vi "Pi_Test_Pulses.vi"(10 "Pi/2 time":dbl=2e-09, 11 "Numeric":i32) -> (3 "x+y":dbl)   [LabVIEW 2024]
panel:
  out "x+y 2":dbl
  in  "clock_freq (MHz)":dbl=500.0
  in  "# of Instructions":u32=3
  in  "Path to spinapi.dll":path=path "C:/SpinCore/SpinAPI/lib/spinapi64.dll"
  in  "Instructions":T1(array[cluster])=[{"Instruct Data"=0, "Op Code"=0, "Flags"=[FALSE, TRUE, TRUE, FALSE, FALSE, FALSE, FALSE, FALSE, FALSE, FALSE, FALSE, FALSE, FALSE, FALSE, FALSE, FALSE, FALSE, FALSE, FALSE, FALSE, FALSE, FALSE, FALSE, TRUE], "Comments"="0", "Time (s)"=1e-07}, {"Instruct Data"=0, "Op Code"=0, "Flags"=[TRUE, TRUE, FALSE, TRUE, FALSE, FALSE, FALSE, FALSE, FALSE, FALSE, FALSE, FALSE, FALSE, FALSE, FALSE, FALSE, FALSE, FALSE, FALSE, FALSE, FALSE, FALSE, FALSE, FALSE], "Comments"="1", "Time (s)"=2e-06}, {"Instruct Data"=0, "Op Code"=6, "Flags"=[FALSE, TRUE, FALSE, FALSE, FALSE, FALSE, FALSE, FALSE, FALSE, FALSE, FALSE, FALSE, FALSE, FALSE, FALSE, FALSE, FALSE, FALSE, FALSE, FALSE, FALSE, FALSE, FALSE, FALSE], "Comments"="2", "Time (s)"=2e-06}, {"Instruct Data"=0, "Op Code"=6, "Flags"=[FALSE, TRUE, FALSE, FALSE, FALSE, FALSE, FALSE, FALSE, FALSE, FALSE, FALSE, FALSE, FALSE, FALSE, FALSE, FALSE, FALSE, FALSE, FALSE, FALSE, FALSE, FALSE, FALSE, FALSE], "Comments"="3", "Time (s)"=2e-06}, {"Instruct Data"=0, "Op Code"=6, "Flags"=[FALSE, TRUE, FALSE, FALSE, FALSE, FALSE, FALSE, FALSE, FALSE, FALSE, FALSE, FALSE, FALSE, FALSE, FALSE, FALSE, FALSE, FALSE, FALSE, FALSE, FALSE, FALSE, FALSE, FALSE], "Comments"="4", "Time (s)"=2e-06}, {"Instruct Data"=0, "Op Code"=6, "Flags"=[FALSE, FALSE, FALSE, FALSE, FALSE, FALSE, FALSE, FALSE, FALSE, FALSE, FALSE, FALSE, FALSE, FALSE, FALSE, FALSE, FALSE, FALSE, FALSE, FALSE, FALSE, FALSE, FALSE, FALSE], "Comments"="5", "Time (s)"=5e-06}, {"Instruct Data"=0, "Op Code"=6, "Flags"=[FALSE, TRUE, TRUE, FALSE, FALSE, FALSE, FALSE, FALSE, FALSE, FALSE, FALSE, FALSE, FALSE, FALSE, FALSE, FALSE, FALSE, FALSE, FALSE, FALSE, FALSE, FALSE, FALSE, FALSE], "Comments"="6", "Time (s)"=3e-06}, {"Instruct Data"=0, "Op Code"=0, "Flags"=[FALSE, TRUE, FALSE, FALSE, FALSE, FALSE, FALSE, FALSE, FALSE, FALSE, FALSE, FALSE, FALSE, FALSE, FALSE, FALSE, FALSE, FALSE, FALSE, FALSE, FALSE, FALSE, FALSE, FALSE], "Comments"="7", "Time (s)"=1e-06}, {"Instruct Data"=0, "Op Code"=0, "Flags"=[FALSE, TRUE, FALSE, FALSE, FALSE, FALSE, FALSE, FALSE, FALSE, FALSE, FALSE, FALSE, FALSE, FALSE, FALSE, FALSE, FALSE, FALSE, FALSE, FALSE, FALSE, FALSE, FALSE, FALSE], "Comments"="8", "Time (s)"=1e-06}, {"Instruct Data"=0, "Op Code"=0, "Flags"=[FALSE, TRUE, FALSE, FALSE, FALSE, FALSE, FALSE, FALSE, FALSE, FALSE, FALSE, FALSE, FALSE, FALSE, FALSE, FALSE, FALSE, FALSE, FALSE, FALSE, FALSE, FALSE, FALSE, FALSE], "Comments"="9", "Time (s)"=1e-06}] {"Time (s)" format="%.3p"; "Op Code" items=["Continue", "Stop", "Loop", "End Loop", "JSR", "RTS", "Branch", "Long Delay", "Wait"]}
  # "1"
  # "2"
  # "3"
  # "4"
  # "5"
  # "6"
  # "7"
  # "8"
  # "9"
  # "10"
  # "11"
  # "12"
  # "13"
  # "14"
  # "15"
  # "16"
  # "17"
  # "18"
  # "19"
  # "20"
  # "21"
  # "22"
  # "23"
  # "24"
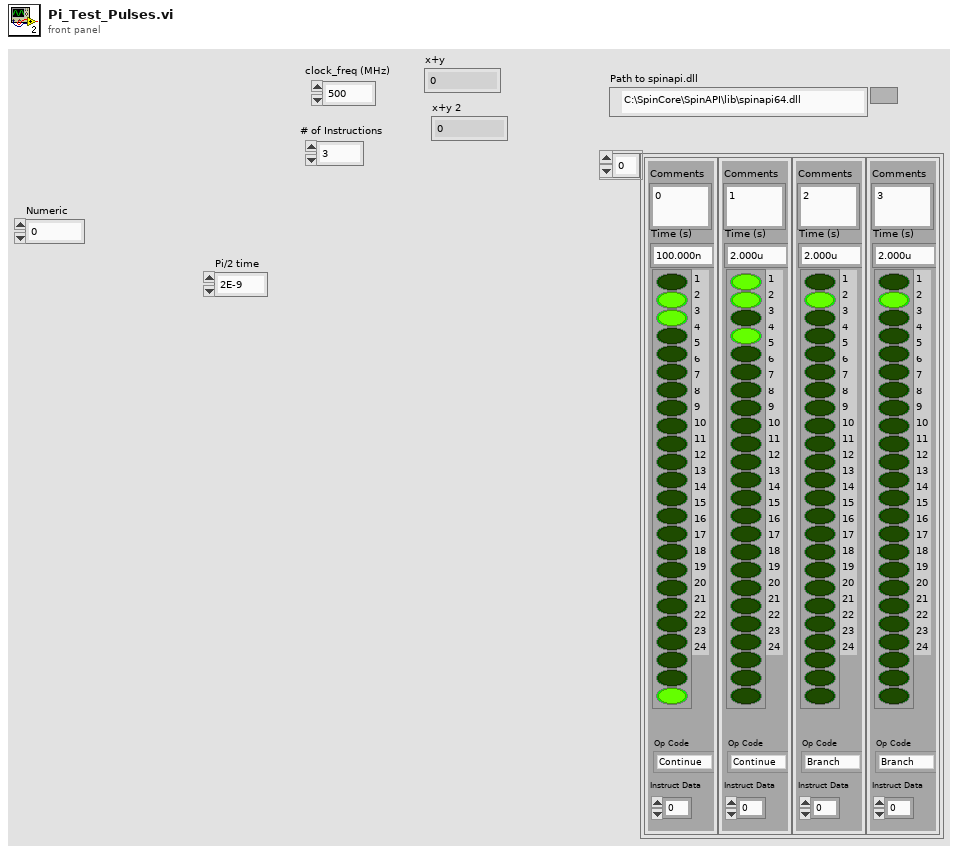
[diagram p1: front panel]
types:
  T1 = cluster{"Instruct Data":i32, "Op Code":i32, "Flags":bool[], "Comments":string, "Time (s)":dbl}[]
  T2 = enum16{"Pulse Program", "Frequency Registers", "TX Phase Registers", "RX Phase Registers"}
  T3 = cluster{"Instruct Data":i32, "Op Code":i32, "Flags":bool[], "Comments":string, "Time (s)":dbl}
  T4 = cluster{"Instruct Data":i32, "Op Code":i32, "Flags":bool[], "Comments":string, dbl}
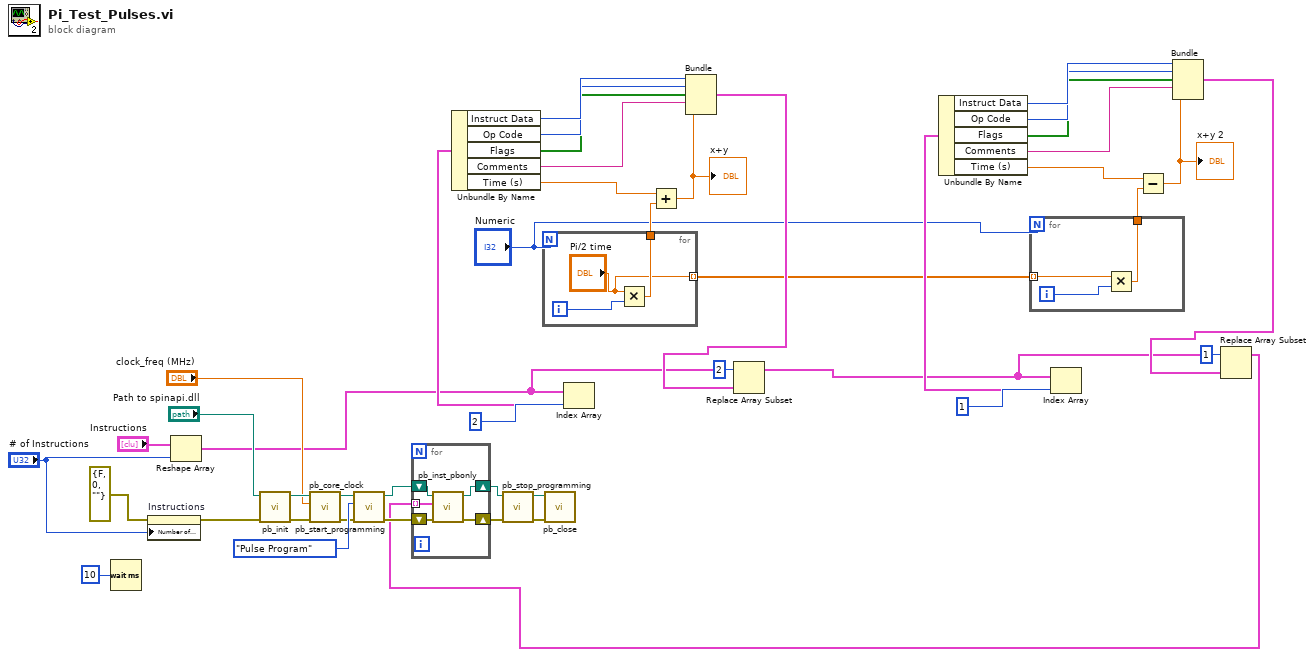
[diagram p0: block diagram]
diagram:
  n1 = Wait (ms)(milliseconds to wait=u32 10) -> ()  [unwired: 1 out]
  n2 = property on="Instructions" class="Arr (strict)"(error in=errorcluster {"status"=FALSE, "code"=0, "source"=""} ("error in (no error)"), "Number of Columns"="# of Instructions") -> (error out=w42:errorcluster)  [unwired: 1 in, 1 out]
  n3 = Reshape Array("Instructions", "# of Instructions") -> (w1:T1)
  n4 = call "pb_init.vi"("error in (no error)"=w42, "path in"="Path to spinapi.dll") -> ("error out"=w35:errorcluster, "path out"=w37:path)  [unwired: 2 in, 6 out]
  n5 = call "pb_core_clock.vi"("error in (no error)"=w35, "clock_freq (MHz)"="clock_freq (MHz)", "path in"=w37) -> ("error out"=w34:errorcluster, "path out"=w36:path)  [unwired: 7 in]
  n6 = call "pb_start_programming.vi"("error in (no error)"=w34, "Device"=T2."Pulse Program", "path in"=w36) -> ("error out"=w40:errorcluster, "path out"=w45:path)  [unwired: 1 in, 6 out]
  n7 = for {
    N: "Numeric" -> [_]
    tunnel: [w47] -> w17
    tunnel: ["Pi/2 time"] -> w3 mode=indexing
    i -> [w48]
    n8 = Multiply(x="Pi/2 time", y=w48) -> (x*y=w47:dbl)
  }
  n9 = Index Array "Index Array"(array=w1, index=2) -> (element=w20:T3)
  n10 = Unbundle By Name "Unbundle By Name"(w20) -> ("Instruct Data"=w26:i32, "Op Code"=w25:i32, "Flags"=w24:bool[], "Comments"=w23:string, "Time (s)"=w22:dbl)
  n11 = Add(x=w22, y=w17) -> (x+y=w21:dbl)
  "x+y" <- w21
  n12 = Bundle("Instruct Data"=w26, "Op Code"=w25, "Flags"=w24, "Comments"=w23, w21) -> (w18:T4)  [unwired: 1 in]
  n13 = Replace Array Subset "Replace Array Subset"(array=w1, new element=w18, index=2) -> (w5:T1)
  n14 = for {
    N: "Numeric" -> [_]
    tunnel: [w50] -> w6
    tunnel: w3 -> [w49] mode=indexing
    i -> [w51]
    n15 = Multiply(x=w49, y=w51) -> (x*y=w50:dbl)
  }
  n16 = Index Array "Index Array"(array=w5, index=1) -> (element=w9:T3)
  n17 = Unbundle By Name "Unbundle By Name"(w9) -> ("Instruct Data"=w15:i32, "Op Code"=w14:i32, "Flags"=w13:bool[], "Comments"=w12:string, "Time (s)"=w11:dbl)
  n18 = Subtract(x=w11, y=w6) -> (x-y=w10:dbl)
  "x+y 2" <- w10
  n19 = Bundle("Instruct Data"=w15, "Op Code"=w14, "Flags"=w13, "Comments"=w12, w10) -> (w7:T4)  [unwired: 1 in]
  n20 = Replace Array Subset "Replace Array Subset"(array=w5, new element=w7, index=1) -> (w2:T1)
  n21 = for {
    tunnel: w2 -> [w53] mode=indexing
    shift-right: [w55] -> w43
    shift-left: w45 -> [w56]
    shift-right: [w52] -> w39
    shift-left: w40 -> [w54]
    n22 = call "pb_inst_pbonly.vi"("error in (no error)"=w54, "PB Instruction"=w53, "path in"=w56) -> ("error out"=w52:errorcluster, "path out"=w55:path)  [unwired: 2 in, 5 out]
  }
  n23 = call "pb_stop_programming.vi"("error in (no error)"=w39, "path in"=w43) -> ("error out"=w38:errorcluster, "path out"=w44:path)  [unwired: 1 in, 7 out]
  n24 = call "pb_close.vi"("error in (no error)"=w38, "path in"=w44) -> ()  [unwired: 10 out]
